vi "Assign Base color and A level.vi"(8 "Data Estimated Info":T3, 10 "S New Info and MiN":T1={"Sample Sequence"="GATGATGATGATGATGAT", "Right Read MIN"=6, "Filter P"=0, "STD Type"=enum."Region", "Base Table"=[], "Selection"=enum."10kHz", "noise MAX"=3, "Sample name"=""} {"Base Table"."Value 3" format="%.2g"}, 11 "Base N info":T2) -> (0 "Color":u32[](array[numeric]), 1 "Base Ex Info":T4, 2 "R Level":dbl[](array[numeric]), 3 "A level":dbl[](array[numeric]))   [LabVIEW 2018]
panel:
  out "STD S level [pA]":dbl[](array[numeric])
  out "G level intensity":dbl
  out "R std":dbl[](array[numeric])
  out "Base S level":dbl[](array[numeric])
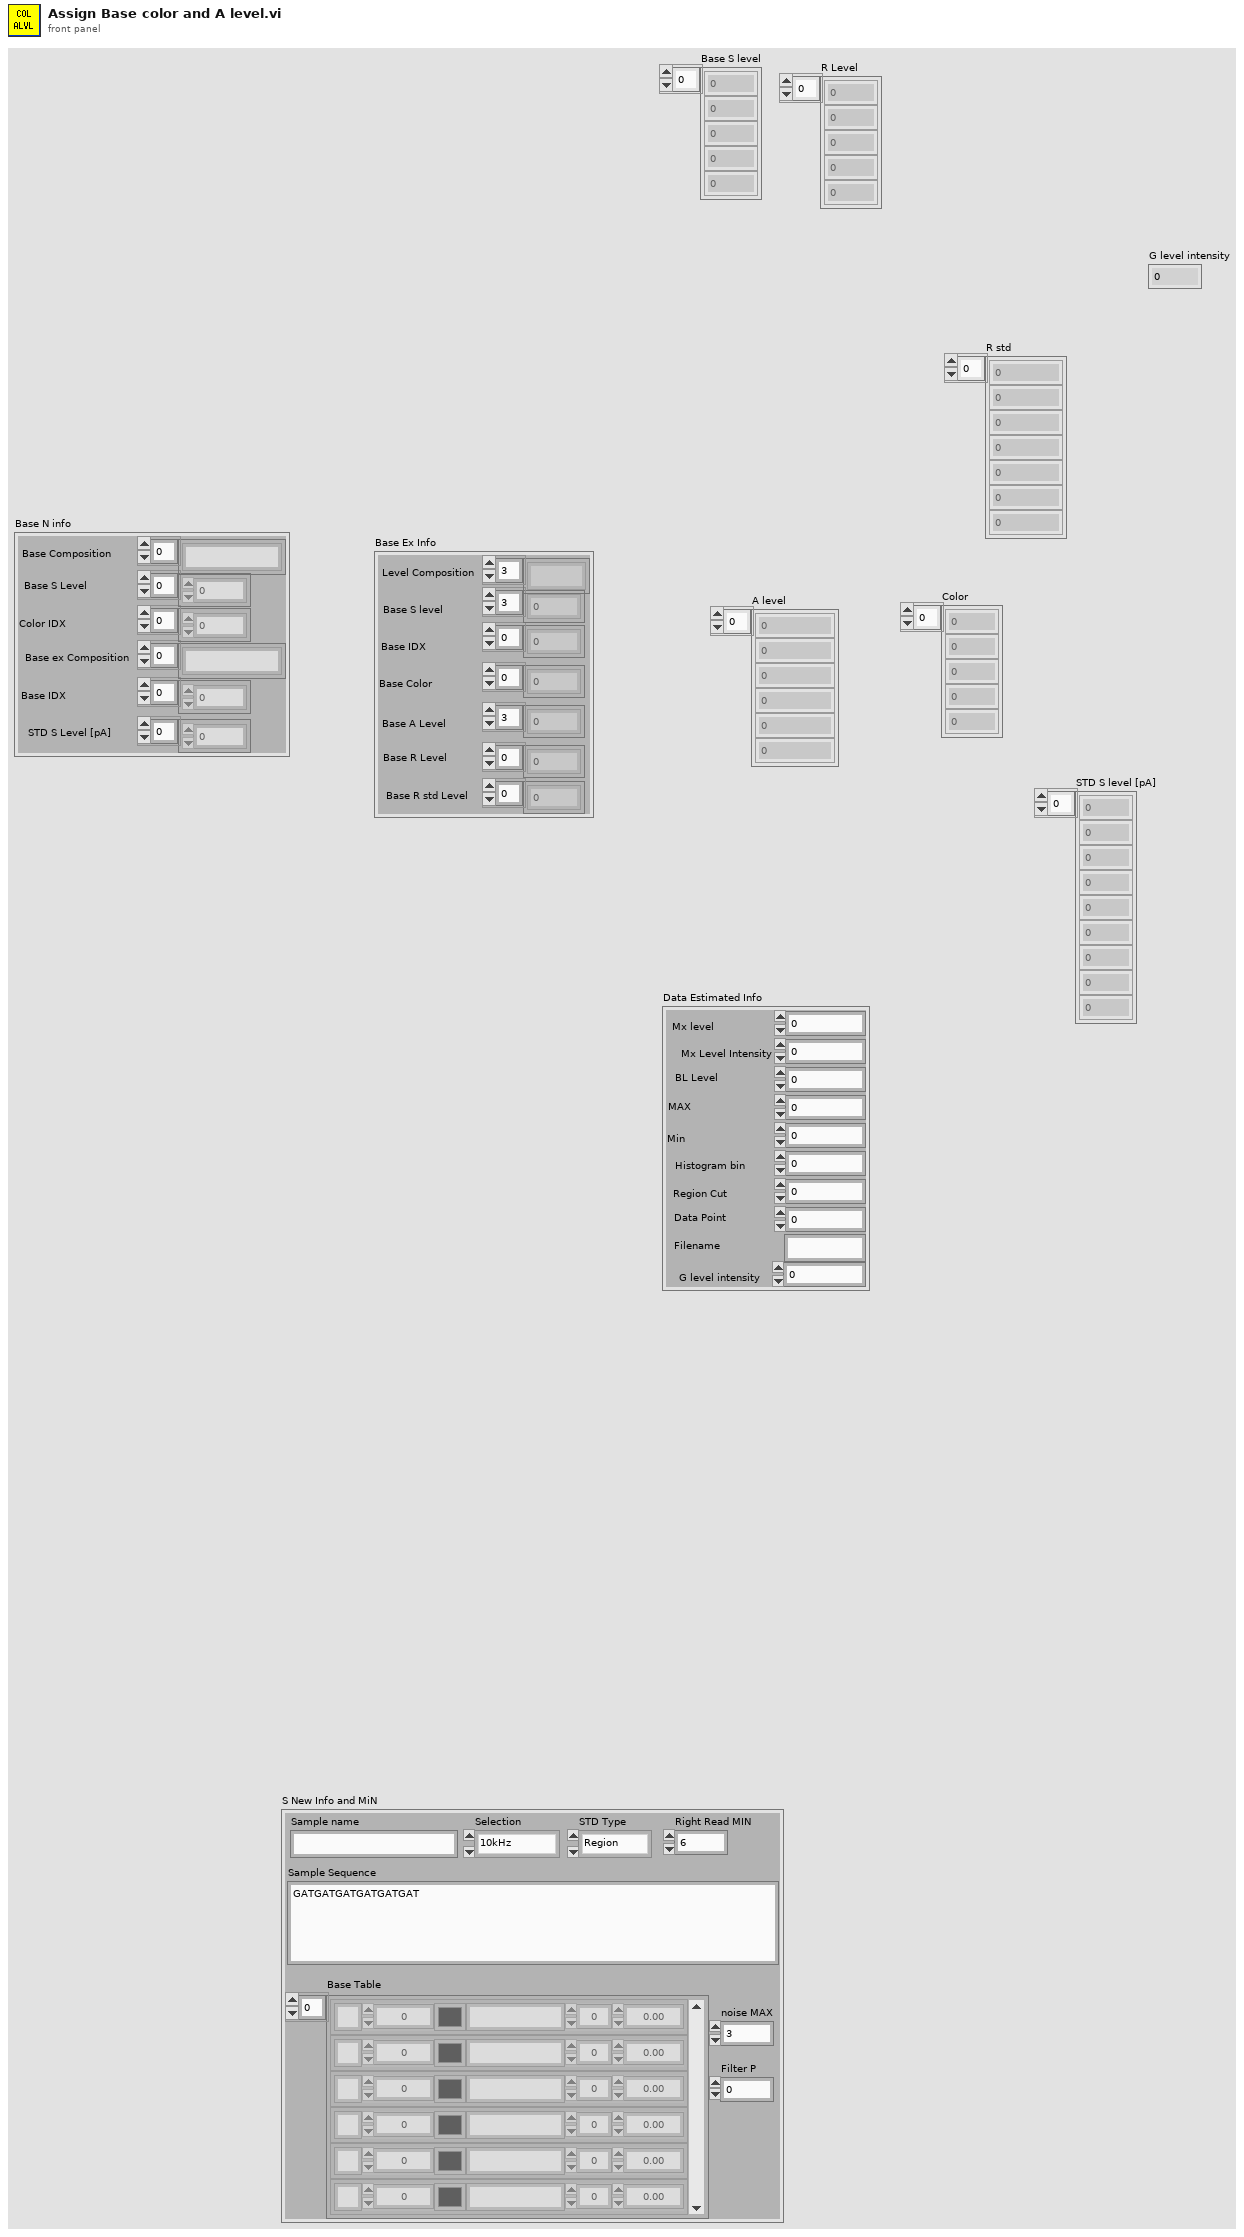
[diagram p1: front panel]
types:
  T1 = cluster{"Sample Sequence":string, "Right Read MIN":i32, "Filter P":i32, "STD Type":enum16{"Region", "Each", "Fixed"}, "Base Table":cluster{"Name":string, "Value":dbl, "Color":u32, "Name 2":string, "Value 2":dbl, "Value 3":dbl}[], "Selection":enum16{"10kHz", "100kHz"}, "noise MAX":i32, "Sample name":string}
  T2 = cluster{"Base Composition":string[], "Base S Level":dbl[], "Color IDX":u32[], "Base ex Composition":string[], "Base IDX":i32[], "STD S Level [pA]":dbl[]}
  T3 = cluster{"Mx level":dbl, "Mx Level Intensity":dbl, "BL Level":dbl, "MAX":dbl, "Min":dbl, "Histogram bin":dbl, "Region Cut":dbl, "Data Point":i32, "Filename":string, "G level intensity":dbl}
  T4 = cluster{"Level Composition":string[], "Base S level":dbl[], "Base IDX":i32[], "Base Color":u32[], "Base A Level":dbl[], "Base R Level":dbl[], "Base R std Level":dbl[]}
  T5 = cluster{"Base Composition":string[], "Base S Level":dbl[], "Base IDX":i32[], "Color IDX":u32[], dbl[], "Base S Level":dbl[], dbl[]}
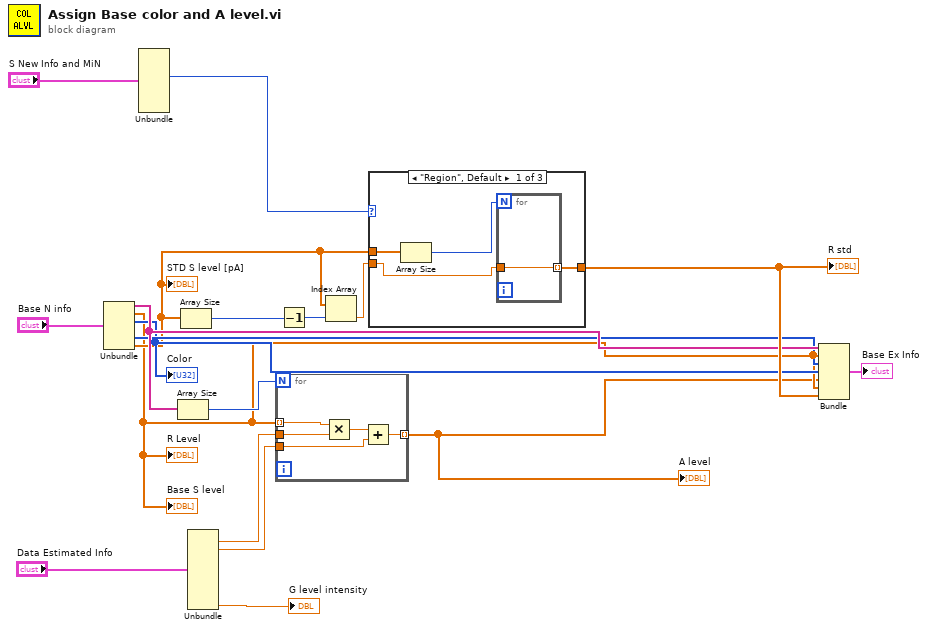
[diagram p0: block diagram]
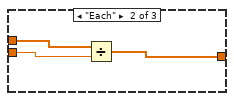
[diagram p2: hidden frame]
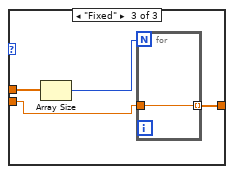
[diagram p3: hidden frame]
diagram:
  n1 = Unbundle("Base N info") -> ("Base Composition"=w11:string[], "Base S Level"=w3:dbl[], "Color IDX"=w8:u32[], "Base IDX"=w10:i32[], "STD S Level [pA]"=w7:dbl[])  [unwired: 1 out]
  "Color" <- w8
  "R Level" <- w3
  "Base S level" <- w3
  "STD S level [pA]" <- w7
  n2 = Unbundle("S New Info and MiN") -> ("STD Type"=w4:enum16{"Region", "Each", "Fixed"})  [unwired: 7 out]
  n3 = Array Size(array=w11) -> (size(s)=w19:i32)
  n4 = Array Size(array=w7) -> (size(s)=w6:i32)
  n5 = Unbundle("Data Estimated Info") -> ("Mx Level Intensity"=w16:dbl, "BL Level"=w18:dbl, "G level intensity"=→"G level intensity":dbl)  [unwired: 7 out]
  n6 = for {
    N: w19 -> [_]
    tunnel: w16 -> [w22]
    tunnel: w18 -> [w23]
    tunnel: [w24] -> w2 mode=indexing
    tunnel: w3 -> [w21] mode=indexing
    n7 = Multiply(x=w21, y=w22) -> (x*y=w20:dbl)
    n8 = Add(x=w20, y=w23) -> (x+y=w24:dbl)
  }
  "A level" <- w2
  n9 = Decrement(x=w6) -> (x-1=w5:i32)
  n10 = Index Array(array=w7, index=w5) -> (element=w1:dbl)
  n11 = case shown="\"Region\", Default" w4 {
    tunnel: w7 -> [w28 w31 w36]
    tunnel: w1 -> [w26 w32 w34]
    tunnel: [w27 w30 w35] -> w13
    frame "Region", Default {
      n12 = Array Size(array=w28) -> (size(s)=w25:i32)
      n13 = for {
        N: w25 -> [_]
        tunnel: w26 -> [w29]
        tunnel: [w29] -> w27 mode=indexing
      }
    }
    frame "Each" {
      n14 = Divide(x=w31, y=w32) -> (x/y=w30:dbl[])
    }
    frame "Fixed" {
      n15 = Array Size(array=w36) -> (size(s)=w33:i32)
      n16 = for {
        N: w33 -> [_]
        tunnel: w34 -> [w37]
        tunnel: [w37] -> w35 mode=indexing
      }
    }
  }
  "R std" <- w13
  n17 = Bundle("Base Composition"=w11, "Base S Level"=w3, "Base IDX"=w10, "Color IDX"=w8, w2, "Base S Level"=w3, w13) -> (→"Base Ex Info":T5)  [unwired: 1 in]
